vi "FuncVI-bgWaveFile.vi"(5 "InstanceRef":T2, 9 "arg list":T1[](array[typedef]) {"num" format="%.2f"}) -> (0 "error out":bool, 3 "result":T1 {"num" format="%.2f"})   [LabVIEW 2021]
doc: "<B>FuncVI-bgWaveFile</B>\n\nThis VI is example of implementation of CalcExpress function (FuncVI). The function reads portion of wave file and returns it as 1D Array of DBL values.\n\n::: CalcExpress Toolkit :::\nCopyright (c) 2000-2026 Konstantin Shifershteyn. All rights reserved."
uses:
  vi.lib/addons/CalcExpress/cetypes.llb/CalcExpress Function Argument Info.ctl
  vi.lib/addons/CalcExpress/cetypes.llb/CalcExpress Instance RefNum.ctl
panel:
  in  "max arg num":i32=4
  in  "min arg num":i32=3
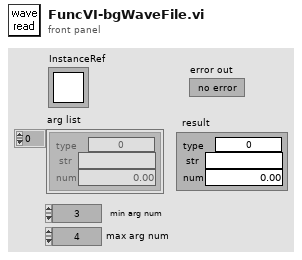
[diagram p1: front panel]
types:
  T1 = typedef "CalcExpress Function Argument Info.ctl" = cluster{"type":u32, "str":string, "num":dbl}
  T2 = typedef "CalcExpress Instance RefNum.ctl" = refnum<k1>
  T3 = enum32{"String", "DBL Number", "identifier", "1D Array of DBL", "2D Array of DBL", "CDB Number", "1D Array of CDB", "2D Array of CDB", "1D Array of String", "2D Array of String", "Unknown data type"}
  T4 = cluster{"index":i32, "data type":enum32{"String", "DBL Number", "identifier", "1D Array of DBL", "2D Array of DBL", "CDB Number", "1D Array of CDB", "2D Array of CDB", "1D Array of String", "2D Array of String", "Unknown data type"}, "default num":dbl, "default str":string}[]
  T5 = cluster{"data type":enum32{"String", "DBL Number", "identifier", "1D Array of DBL", "2D Array of DBL", "CDB Number", "1D Array of CDB", "2D Array of CDB", "1D Array of String", "2D Array of String", "Unknown data type"}, "data string":string, dbl}
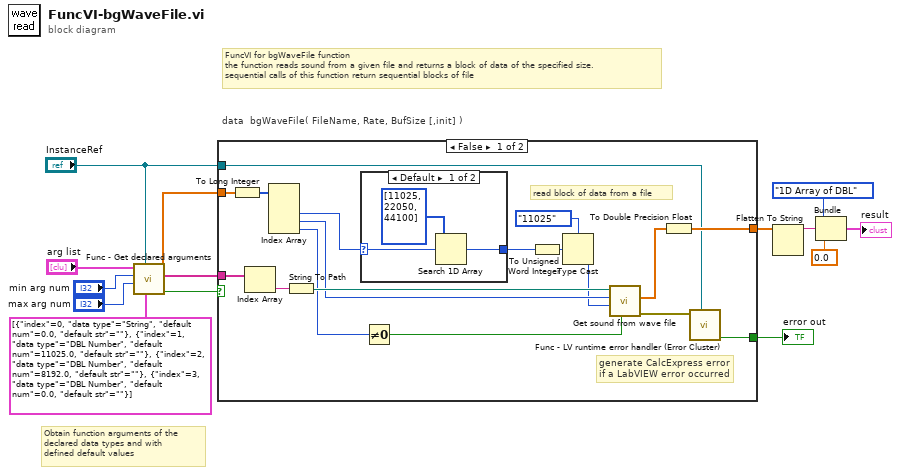
[diagram p0: block diagram]
diagram:
  # "FuncVI for bgWaveFile function\nthe function reads sound from a given file and returns a block of data of the specified size.\nsequential calls of this function return sequential blocks of file"
  # "Obtain function arguments of the\ndeclared data types and with\ndefined default values"
  # "data  bgWaveFile( FileName, Rate, BufSize [,init] )"
  n1 = call "Func - Get declared arguments.vi"("arg descriptors"=T4 [{"index"=0, "data type"=enum."String", "default num"=0.0, "default str"=""}, {"index"=1, "data type"=enum."DBL Number", "default num"=11025.0, "default str"=""}, {"index"=2, "data type"=enum."DBL Number", "default num"=8192.0, "default str"=""}, {"index"=3, "data type"=enum."DBL Number", "default num"=0.0, "default str"=""}] ("args descriptors"), "InstanceRef"="InstanceRef", "max arg num"="max arg num", "min arg num"="min arg num", "arg list"="arg list") -> ("error out"=w10:bool, "str list"=w1:string[], "num list"=w7:dbl[])  [unwired: 3 in, 1 out]
  n2 = case shown="False" w10 {
    selector: w10 -> [_ w37]
    tunnel: [w28 _] -> w9
    tunnel: [w25 w37] -> w4
    tunnel: "InstanceRef" -> [w26 _]
    tunnel: w7 -> [w31 _]
    tunnel: w1 -> [w24 _]
    frame False {
      # "read block of data from a file"
      # "generate CalcExpress error\nif a LabVIEW error occurred"
      n3 = To Long Integer(number=w31) -> (32bit integer=w22:i32[])
      n4 = Index Array(array=w24) -> (element=w23:string)  [unwired: 1 in]
      n5 = Index Array(array=w22) -> (element #2=w16:i32, element #3=w20:i32, element #4=w21:i32)  [unwired: 4 in, 1 out]
      n6 = String To Path(string=w23) -> (path=w32:path)
      n7 = case shown="Default" w16 {
        selector: w16 -> [w34 w36]
        tunnel: [w33 w36] -> w15
        frame Default {
          n8 = Search 1D Array(1D array=i32[] [11025, 22050, 44100], element=w34) -> (index of element=w33:i32)  [unwired: 1 in]
        }
        frame 0..2 {
        }
      }
      n9 = Not Equal To 0?(x=w21) -> (x != 0?=w30:bool)
      n10 = To Unsigned Word Integer(number=w15) -> (unsigned 16bit integer=w19:u16)
      n11 = Type Cast(type=enum16{"11025", "22050", "44100"}."11025" ("Sound Rate"), x=w19) -> (*(type *) &x=w17:enum16{"11025", "22050", "44100"})
      n12 = call "Get sound from wave file.vi"("init"=w30, "Sound Rate"=w17, "buffer size (samples)"=w20, "wave file"=w32) -> ("error out"=w27:errorcluster, "sound portion"=w29:dbl[])  [unwired: 3 in, 3 out]
      n13 = To Double Precision Float(number=w29) -> (double precision float=w28:dbl[])
      n14 = call "Func - LV runtime error handler (Error Cluster).vi"("InstanceRef"=w26, "LabVIEW error"=w27) -> ("error out"=w25:bool)  [unwired: 4 in, 3 out]
    }
    frame True {
    }
  }
  "error out" <- w4
  n15 = Flatten To String(anything=w9) -> (data string=w6:string)  [unwired: 3 in, 2 out]
  n16 = Bundle("data type"=T3."1D Array of DBL", "data string"=w6, 0.0) -> (→"result":T5)  [unwired: 1 in]
